vi "Format HW label name.vi"(7 "Use Octal Channel Names?":bool, 8 "formatting":enum16{"NIVeriStandAdd-Ons", "ni"}(ring), 9 "Label Name in":string, 10 "SDI":i32, 11 "Label Decimal":u32) -> (3 "Label Name out":string)   [LabVIEW 2020]
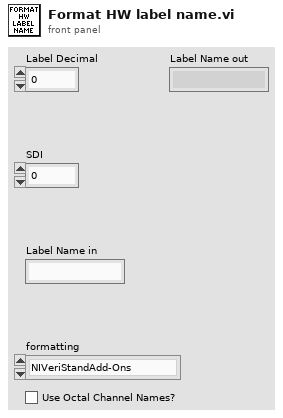
[diagram p1: front panel]
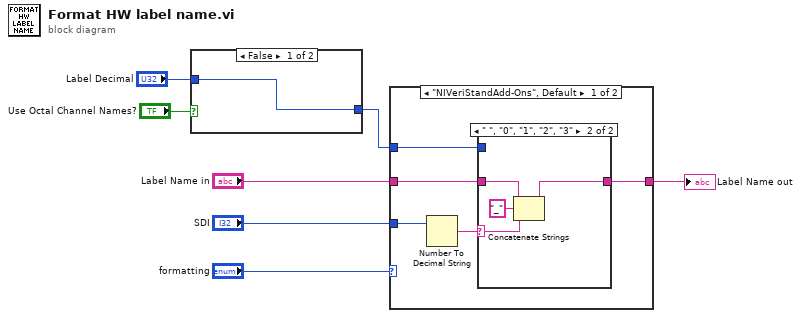
[diagram p0: block diagram]
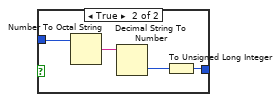
[diagram p2: hidden frame]
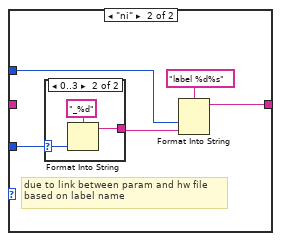
[diagram p4: hidden frame]
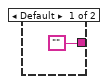
[diagram p5: hidden frame]
diagram:
  n1 = case shown="False" "Use Octal Channel Names?" {
    tunnel: [w8 w10] -> w1
    tunnel: "Label Decimal" -> [w8 w11]
    frame False {
    }
    frame True {
      n2 = Number To Octal String(2:w11) -> (0:w12:string)  [unwired: 1 in]
      n3 = Decimal String To Number(string=w12) -> (number=w9:i32)  [unwired: 2 in, 1 out]
      n4 = To Unsigned Long Integer(number=w9) -> (unsigned 32bit integer=w10:u32)
    }
  }
  n5 = case shown="\"NIVeriStandAdd-Ons\", Default" "formatting" {
    tunnel: [w13 w25] -> w4
    tunnel: "Label Name in" -> [w16 _]
    tunnel: "SDI" -> [w15 w24]
    tunnel: w1 -> [w14 w26]
    frame "NIVeriStandAdd-Ons", Default {
      n6 = Number To Decimal String(number=w15) -> (decimal integer string=w17:string)  [unwired: 1 in]
      n7 = case shown="\" \", \"0\", \"1\", \"2\", \"3\"" w17 {
        selector: w17 -> [_ w19]
        tunnel: w16 -> [w18 w22]
        tunnel: [w18 w20] -> w13
        tunnel: w14 -> [_ _]
        frame "False", Default {
        }
        frame " ", "0", "1", "2", "3" {
          n8 = Concatenate Strings(w22, "_" ("string"), w19) -> (w20:string)
        }
      }
    }
    frame "ni" {
      # "due to link between param and hw file\nbased on label name"
      n9 = case shown="0..3" w24 {
        selector: w24 -> [_ w30]
        tunnel: ["" w29] -> w23
        frame Default {
        }
        frame 0..3 {
          n10 = Format Into String(format string="_%d", w30) -> (resulting string=w29:string)  [unwired: 2 in, 1 out]
        }
      }
      n11 = Format Into String(format string="label %d%s", w26, w23) -> (resulting string=w25:string)  [unwired: 2 in, 1 out]
    }
  }
  "Label Name out" <- w4
